vi "PicoScope5000aGetTimebase2.vi"(4 "Number of Samples":u32, 6 "Memory Segment":u32, 7 "Acquisition Settings":T2 {"postTriggerSamples" format="%_6p"; "preTriggerSamples" format="%_6p"}, 10 "handle in":i16, 11 "error in (no error)":errorcluster) -> (2 "handle out":i16, 3 "error out":errorcluster, 5 "Properties Panel":T1 {"Max Total Capture Time Available (sec)" format="%.3p"; "Sample Frequency" format="%.3p"; "Sample Rate" format="%.3p"; "Max Samples Available" format="%.3p"; "Total Capture Time (sec)" format="%.3p"})   [LabVIEW 2009]
uses:
  ps5000a.dll
  shared/Acquisition Settings.ctl
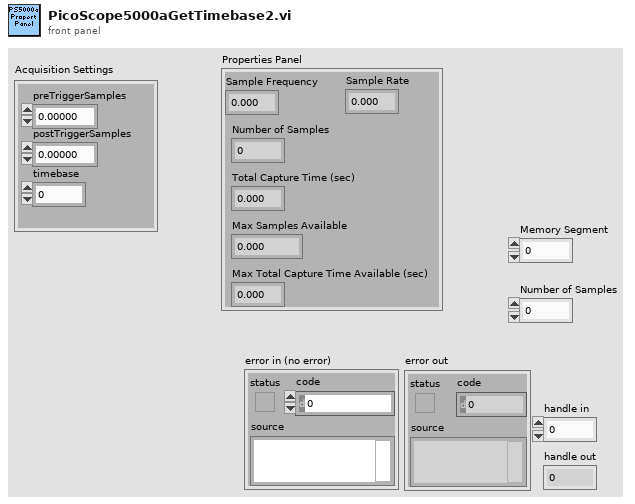
[diagram p1: front panel]
types:
  T1 = cluster{"Sample Frequency":sgl, "Sample Rate":sgl, "Max Samples Available":i32, "Number of Samples":u32, "Total Capture Time (sec) ":sgl, "Max Total Capture Time Available (sec)":sgl}
  T2 = typedef "Acquisition Settings.ctl" = cluster{"preTriggerSamples":u64, "postTriggerSamples":u64, "timebase":u32}
  T3 = cluster{sgl, sgl, "maxSamples":i32, "Number of Samples":u32, sgl, sgl}
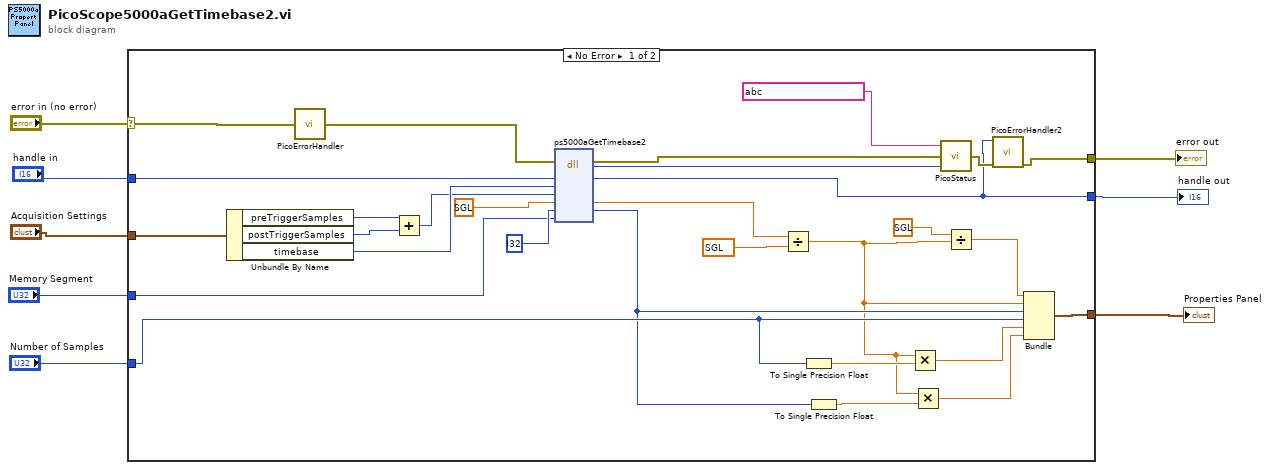
[diagram p0: block diagram]
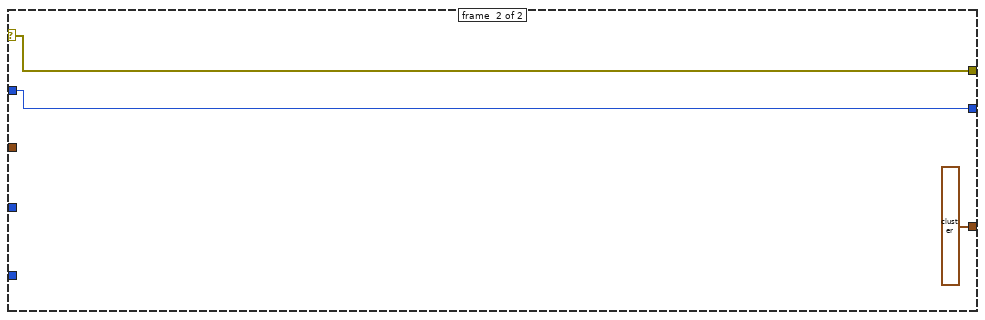
[diagram p2: hidden frame]
diagram:
  n1 = case shown="No Error" "error in (no error)" {
    selector: "error in (no error)" -> [w27 w40]
    tunnel: [w11 w40] -> w8
    tunnel: [w9 w39] -> w7
    tunnel: "Memory Segment" -> [w26 _]
    tunnel: "Number of Samples" -> [w20 _]
    tunnel: "handle in" -> [w25 w39]
    tunnel: "Acquisition Settings" -> [w24 _]
    tunnel: [w16 T3 ?] -> w1
    frame #0 {
      n2 = Unbundle By Name(w24) -> ("preTriggerSamples"=w31:u64, "postTriggerSamples"=w32:u64, "timebase"=w33:u32)
      n3 = call "PicoErrorHandler.vi"("error in"=w27) -> ("error out"=w35:errorcluster)
      n4 = Add(x=w31, y=w32) -> (x+y=w22:u64)
      n5 = dll-call lib="ps5000a.dll" fn="ps5000aGetTimebase2"(error in=w35, "handle"=w25, "timebase"=w33, "noSamples"=w22, "timeIntervalNanoseconds"=sgl ?, "maxSamples"=i32 ?, "segmentIndex"=w26) -> (error out=w34:errorcluster, "PICO_STATUS"=w10:u32, "handle"=w9:i16, "timeIntervalNanoseconds"=w36:sgl, "maxSamples"=w18:i32)  [unwired: 5 in, 1 out]
      n6 = Divide(x=w36, y=sgl ?) -> (x/y=w15:sgl)
      n7 = To Single Precision Float(number=w20) -> (single precision float=w23:sgl)
      n8 = To Single Precision Float(number=w18) -> (single precision float=w19:sgl)
      n9 = Multiply(x=w15, y=w23) -> (x*y=w21:sgl)
      n10 = Multiply(x=w15, y=w19) -> (x*y=w17:sgl)
      n11 = call "PicoStatus.vi"("PICO STATUS"=w10, "error in"=w34, "source"=string ?) -> ("error out"=w12:errorcluster)
      n12 = Divide(x=sgl ?, y=w15) -> (x/y=w13:sgl)
      n13 = call "PicoErrorHandler2.vi"("error in (no error)"=w12, "handle In"=w9) -> ("error out"=w11:errorcluster)  [unwired: 9 in]
      n14 = Bundle(w13, w15, "maxSamples"=w18, "Number of Samples"=w20, w21, w17) -> (w16:T3)  [unwired: 1 in]
    }
    frame #1 {
    }
  }
  "error out" <- w8
  "handle out" <- w7
  "Properties Panel" <- w1
